vi "[ce] State Queue Parser.vi"(9 "input queue":string) -> (0 "state parameters":string, 2 "state":string, 3 "remained queue":string)   [LabVIEW 2021]
doc: "The VI extracts and parses the first state specifier from a State Queue represented as a string with the syntax described below. A state queue can consists of zero or more state specifiers.\n\nA syntax of state specifier:\n State [ = parameters] ;\n, where\n1) State is a keyword specifying a state be performed.\n2) Parameters is an optional sub-string. It must start with an equality sign (can be surrounded by spaces). Parameters sub-string cannot contain semicolons, all the other characters are allowed.\n3) Semicolon is a delimiter of a state specifier. Semicolon can be surrounded by CR,LF and Space characters\n\nExamples:\n1) Show Help;\n2) Save File = filepath;\n3) DoSomething=param1; DoSomething=param2; All Done;\n\n::: CalcExpress Toolkit :::\nCopyright (c) 2000-2026 Konstantin Shifershteyn. All rights reserved."
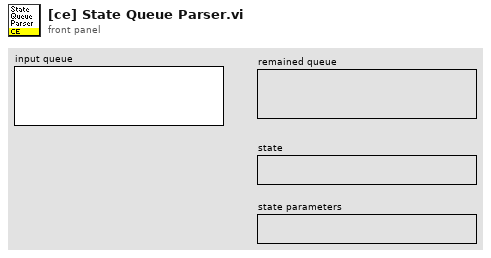
[diagram p1: front panel]
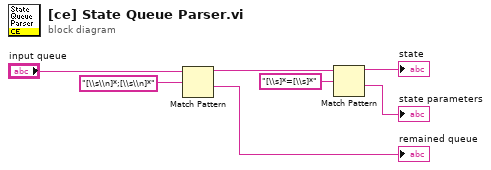
[diagram p0: block diagram]
diagram:
  n1 = Match Pattern(string="input queue", regular expression="[\\s\\n]*;[\\s\\n]*") -> (before substring=w6:string, after substring=→"remained queue":string)  [unwired: 3 out]
  n2 = Match Pattern(string=w6, regular expression="[\\s]*=[\\s]*") -> (before substring=→"state":string, after substring=→"state parameters":string)  [unwired: 3 out]
